vi "Read Modbus_Master.lvclass.vi"(8 "error in (no error)":errorcluster, 11 "Modbus_AO in":refnum<class "Modbus_AO.lvclass">) -> (0 "error out":errorcluster, 2 "Modbus_Master.lvclass":refnum<class "Modbus_Master.lvclass">, 3 "Modbus_AO out":refnum<class "Modbus_AO.lvclass">)   [LabVIEW 2021, in "Modbus_AO.lvclass"]
uses:
  Modbus_AO.lvclass
  Modbus_Master/Modbus_Master.lvclass
  Modbus_AO.lvclass/Modbus_AO.ctl
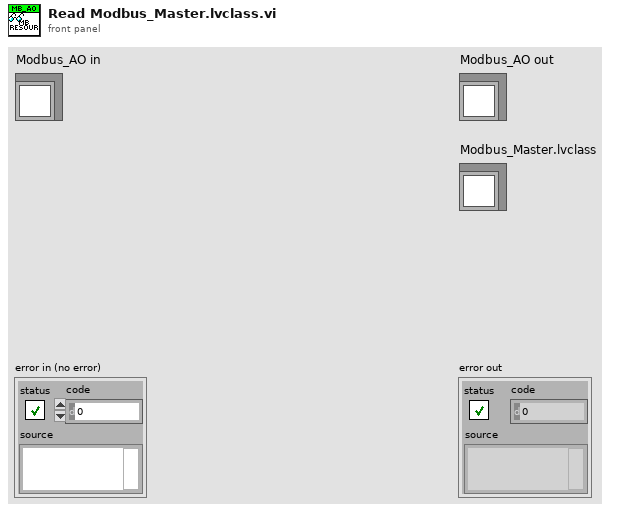
[diagram p1: front panel]
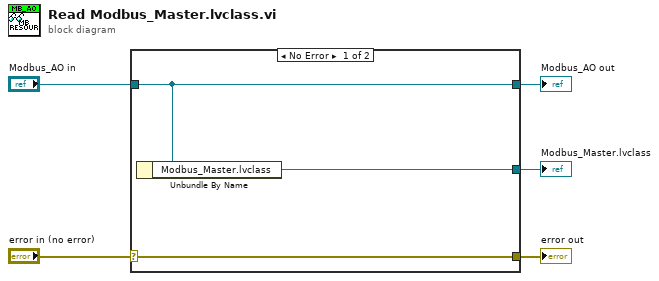
[diagram p0: block diagram]
diagram:
  n1 = case shown="No Error" "error in (no error)" {
    selector: "error in (no error)" -> [w8 w9]
    tunnel: [w8 w9] -> w4
    tunnel: [w7 w10] -> w2
    tunnel: "Modbus_AO in" -> [w7 w10]
    tunnel: [w6 _] -> w1
    frame No Error {
      n2 = Unbundle By Name(w7) -> ("Modbus_Master.lvclass"=w6:refnum<class "Modbus_Master.lvclass">)
    }
    frame Error {
    }
  }
  "error out" <- w4
  "Modbus_AO out" <- w2
  "Modbus_Master.lvclass" <- w1
